vi "Rule_Check_Forbidden.vi"(8 "error in":errorcluster, 9 "Renju":bool=TRUE, 10 "Move":T2={"Row"=7, "Col"=7, "Stone"=enum."Black"}, 11 "Grid":enum8{"Empty", "Black", "White"}[][](array[ring])=[[enum."Empty", enum."Empty", enum."Empty", enum."Empty", enum."Empty", enum."Empty", enum."Empty", enum."Empty", enum."Empty", enum."Empty", enum."Empty", enum."Empty", enum."Empty", enum."Empty", enum."Empty"], [enum."Empty", enum."Empty", enum."Empty", enum."Empty", enum."Empty", enum."Empty", enum."Empty", enum."Empty", enum."Empty", enum."Empty", enum."Empty", enum."Empty", enum."Empty", enum."Empty", enum."Empty"], [enum."Empty", enum."Empty", enum."Empty", enum."Empty", enum."Empty", enum."Empty", enum."Empty", enum."Empty", enum."Empty", enum."Empty", enum."Empty", enum."Empty", enum."Empty", enum."Empty", enum."Empty"], [enum."Empty", enum."Empty", enum."Empty", enum."Empty", enum."Empty", enum."Empty", enum."Empty", enum."Empty", enum."Empty", enum."Empty", enum."Empty", enum."Empty", enum."Empty", enum."Empty", enum."Empty"], [enum."Empty", enum."Empty", enum."Empty", enum."Empty", enum."Empty", enum."Empty", enum."Empty", enum."Empty", enum."Empty", enum."Empty", enum."Empty", enum."Empty", enum."Empty", enum."Empty", enum."Empty"], [enum."Empty", enum."Empty", enum."Empty", enum."Empty", enum."Empty", enum."Empty", enum."Empty", enum."Empty", enum."Empty", enum."Empty", enum."Empty", enum."Empty", enum."Empty", enum."Empty", enum."Empty"], [enum."Empty", enum."Empty", enum."Empty", enum."Empty", enum."Empty", enum."Empty", enum."Empty", enum."Empty", enum."Empty", enum."Empty", enum."Empty", enum."Empty", enum."Empty", enum."Empty", enum."Empty"], [enum."Empty", enum."Empty", enum."Empty", enum."Empty", enum."Empty", enum."Empty", enum."Empty", enum."Empty", enum."Empty", enum."Empty", enum."Empty", enum."Empty", enum."Empty", enum."Empty", enum."Empty"], [enum."Empty", enum."Empty", enum."Empty", enum."Empty", enum."Empty", enum."Empty", enum."Empty", enum."Empty", enum."Empty", enum."Empty", enum."Empty", enum."Empty", enum."Empty", enum."Empty", enum."Empty"], [enum."Empty", enum."Empty", enum."Empty", enum."Empty", enum."Empty", enum."Empty", enum."Empty", enum."Empty", enum."Empty", enum."Empty", enum."Empty", enum."Empty", enum."Empty", enum."Empty", enum."Empty"], [enum."Empty", enum."Empty", enum."Empty", enum."Empty", enum."Empty", enum."Empty", enum."Empty", enum."Empty", enum."Empty", enum."Empty", enum."Empty", enum."Empty", enum."Empty", enum."Empty", enum."Empty"], [enum."Empty", enum."Empty", enum."Empty", enum."Empty", enum."Empty", enum."Empty", enum."Empty", enum."Empty", enum."Empty", enum."Empty", enum."Empty", enum."Empty", enum."Empty", enum."Empty", enum."Empty"], [enum."Empty", enum."Empty", enum."Empty", enum."Empty", enum."Empty", enum."Empty", enum."Empty", enum."Empty", enum."Empty", enum."Empty", enum."Empty", enum."Empty", enum."Empty", enum."Empty", enum."Empty"], [enum."Empty", enum."Empty", enum."Empty", enum."Empty", enum."Empty", enum."Empty", enum."Empty", enum."Empty", enum."Empty", enum."Empty", enum."Empty", enum."Empty", enum."Empty", enum."Empty", enum."Empty"], [enum."Empty", enum."Empty", enum."Empty", enum."Empty", enum."Empty", enum."Empty", enum."Empty", enum."Empty", enum."Empty", enum."Empty", enum."Empty", enum."Empty", enum."Empty", enum."Empty", enum."Empty"]]) -> (0 "error out":errorcluster, 2 "Reason":T1(ring), 3 "Forbidden?":bool)   [LabVIEW 2026]
doc: "렌주룰 흑 금수 판정(3-3, 4-4, 장목). 흑을 가상 착수한 뒤 4방향 연속 수를 본다.\n단순화: 연속된 돌만 판정(띈 3/띈 4 미포함), 거짓 금수 재귀 판정 없음. 정확히 5목이면 금수 아님."
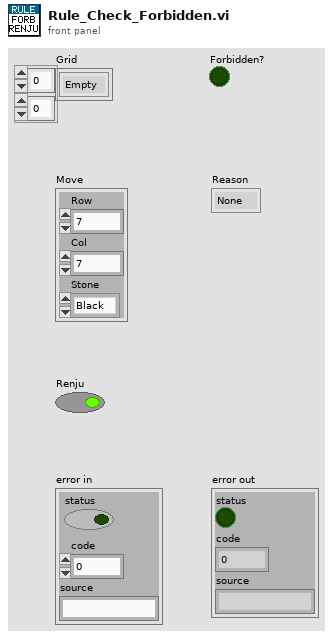
[diagram p1: front panel]
types:
  T1 = enum8{"None", "Double Three", "Double Four", "Overline"}
  T2 = cluster{"Row":i32, "Col":i32, "Stone":enum8{"Empty", "Black", "White"}}
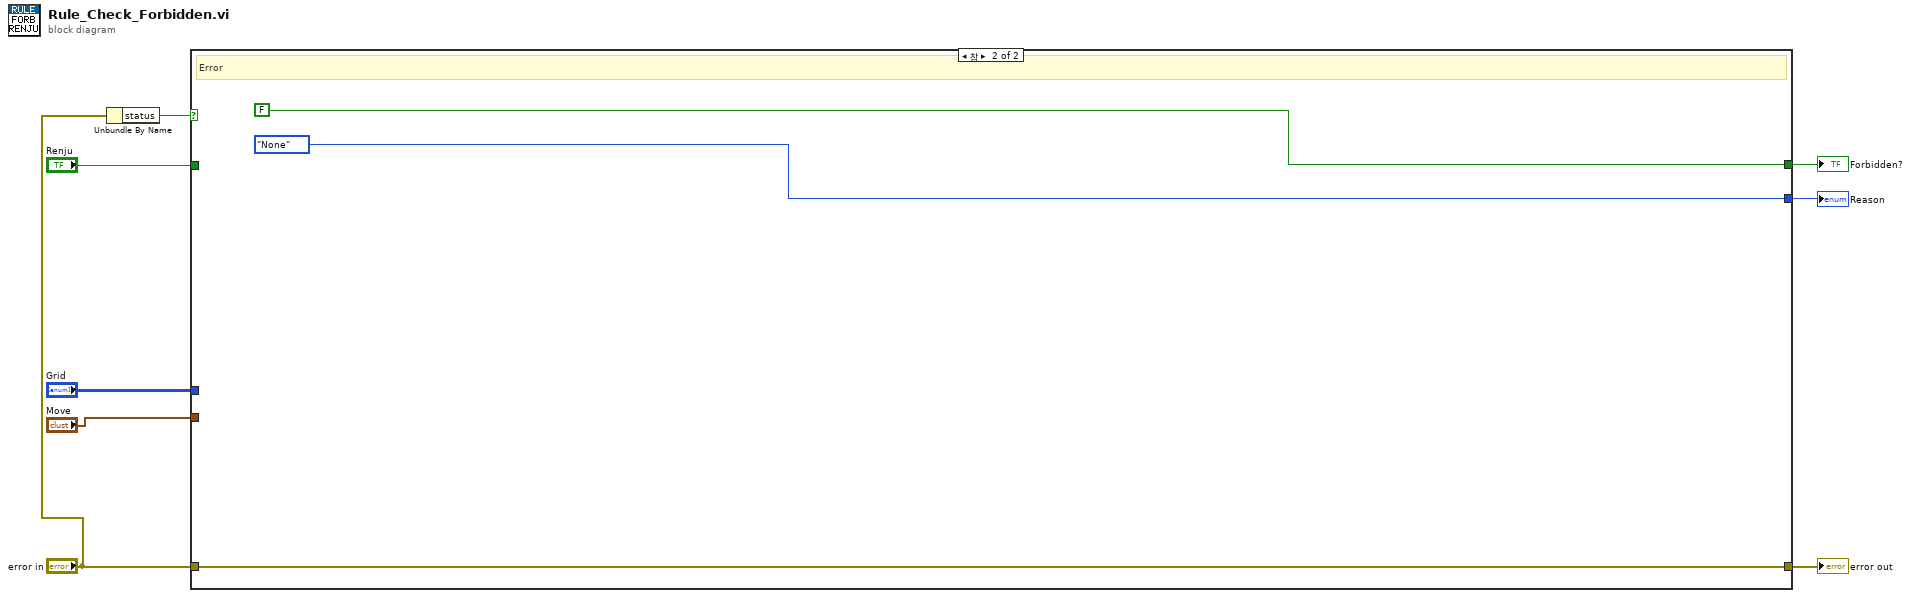
[diagram p0: block diagram]
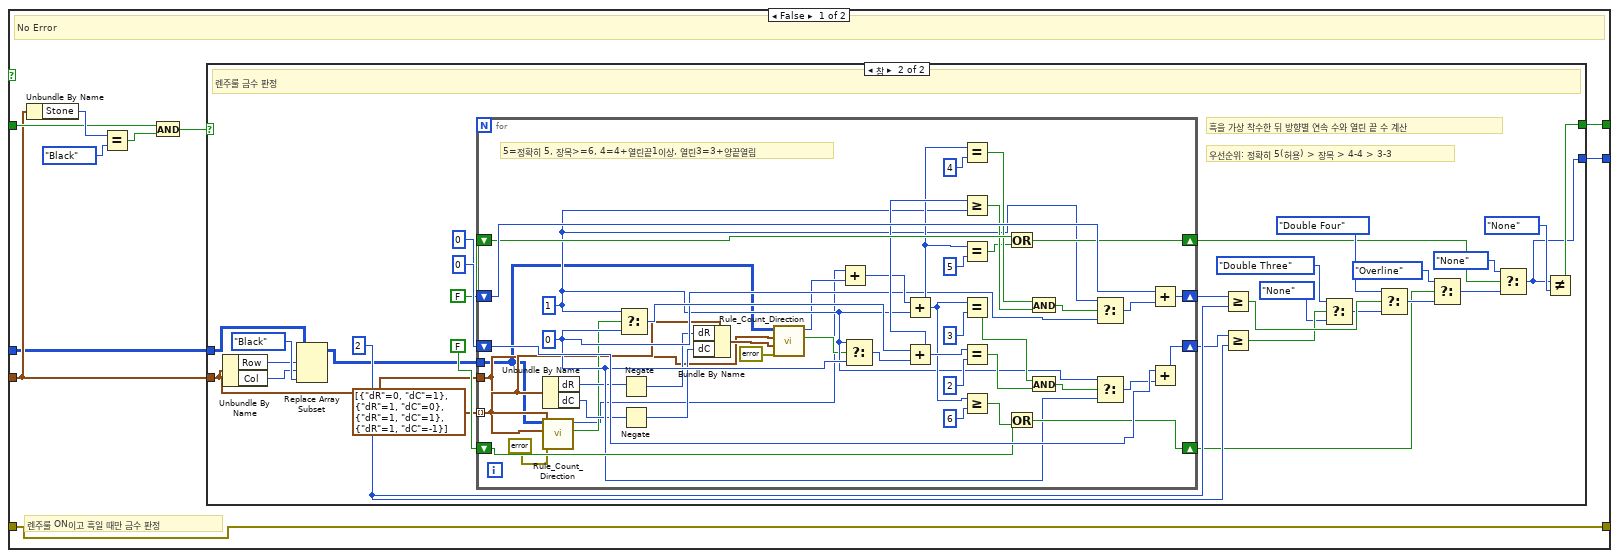
[diagram p2: hidden frame]
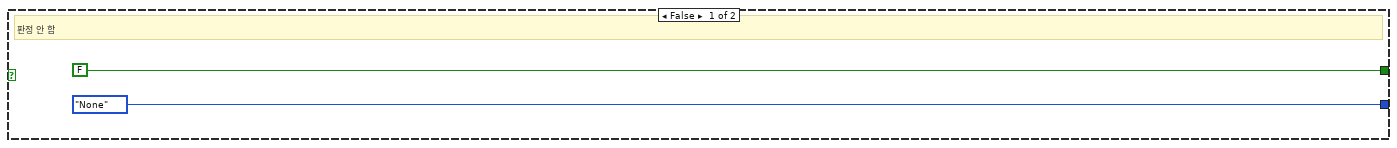
[diagram p3: hidden frame]
diagram:
  n1 = Unbundle By Name("error in") -> ("status"=w5:bool)
  n2 = case shown="참" w5 {
    tunnel: "Grid" -> [w9 _]
    tunnel: "Move" -> [w10 _]
    tunnel: "Renju" -> [w11 _]
    tunnel: "error in" -> [w12 w94]
    tunnel: [w12 w94] -> w8
    tunnel: [w18 T1."None"] -> w7
    tunnel: [w17 FALSE] -> w6
    frame False {
      # "렌주룰 ON이고 흑일 때만 금수 판정"
      # "No Error"
      n3 = Unbundle By Name(w10) -> ("Stone"=w13:enum8{"Empty", "Black", "White"})
      n4 = Equal?(x=w13, y=enum8{"Empty", "Black", "White"}."Black") -> (x = y?=w15:bool)
      n5 = And(x=w11, y=w15) -> (x .and. y?=w16:bool)
      n6 = case shown="참" w16 {
        tunnel: w9 -> [_ w21]
        tunnel: w10 -> [_ w22]
        tunnel: [T1."None" w47] -> w18
        tunnel: [FALSE w49] -> w17
        frame False {
          # "판정 안 함"
        }
        frame True {
          w36 = 2
          # "우선순위: 정확히 5(허용) > 장목 > 4-4 > 3-3"
          # "흑을 가상 착수한 뒤 방향별 연속 수와 열린 끝 수 계산"
          # "렌주룰 금수 판정"
          n7 = Unbundle By Name(w22) -> ("Row"=w23:i32, "Col"=w24:i32)
          n8 = Replace Array Subset(array=w21, new element=enum8{"Empty", "Black", "White"}."Black", index (row)=w23, index (col)=w24) -> (w26:enum8{"Empty", "Black", "White"}[][])
          n9 = for {
            tunnel: cluster{"dR":i32, "dC":i32}[] [{"dR"=0, "dC"=1}, {"dR"=1, "dC"=0}, {"dR"=1, "dC"=1}, {"dR"=1, "dC"=-1}] ("Directions") -> [w52] mode=indexing
            shift-right: [w84] -> w32
            shift-left: FALSE -> [w85]
            shift-right: [w86] -> w33
            shift-left: FALSE -> [w87]
            shift-right: [w89] -> w34
            shift-left: 0 -> [w90]
            shift-right: [w92] -> w35
            shift-left: 0 -> [w93]
            tunnel: w22 -> [w51]
            tunnel: w26 -> [w50]
            w65 = 0
            w64 = 1
            # "5=정확히 5, 장목>=6, 4=4+열린끝1이상, 열린3=3+양끝열림"
            n10 = Unbundle By Name(w52) -> ("dR"=w56:i32, "dC"=w57:i32)
            n11 = call "Rule_Count_Direction.vi"("error in"=errorcluster {"status"=FALSE, "code"=0, "source"=""}, "Direction"=w52, "Move"=w51, "Grid"=w50) -> ("Open End"=w55:bool, "Count"=w54:i32)  [unwired: 5 in, 1 out]
            n12 = Select(t=w64, s=w55, f=w65) -> (s? t:f=w68:i32)
            n13 = Negate(x=w56) -> (-x=w58:i32)
            n14 = Negate(x=w57) -> (-x=w59:i32)
            n15 = Bundle By Name(cluster=w52, "dR"=w58, "dC"=w59) -> (w60:cluster{"dR":i32, "dC":i32})
            n16 = call "Rule_Count_Direction.vi"("error in"=errorcluster {"status"=FALSE, "code"=0, "source"=""}, "Direction"=w60, "Move"=w51, "Grid"=w50) -> ("Open End"=w63:bool, "Count"=w62:i32)  [unwired: 5 in, 1 out]
            n17 = Add(x=w54, y=w62) -> (x+y=w66:i32)
            n18 = Select(t=w64, s=w63, f=w65) -> (s? t:f=w69:i32)
            n19 = Add(x=w66, y=w64) -> (x+y=w67:i32)
            n20 = Add(x=w68, y=w69) -> (x+y=w70:i32)
            n21 = Equal?(x=w67, y=4) -> (x = y?=w76:bool)
            n22 = Greater Or Equal?(x=w70, y=w64) -> (x >= y?=w77:bool)
            n23 = Equal?(x=w67, y=5) -> (x = y?=w72:bool)
            n24 = Equal?(x=w67, y=3) -> (x = y?=w80:bool)
            n25 = Equal?(x=w70, y=2) -> (x = y?=w82:bool)
            n26 = Greater Or Equal?(x=w67, y=6) -> (x >= y?=w74:bool)
            n27 = Or(x=w85, y=w72) -> (x .or. y?=w84:bool)
            n28 = Or(x=w87, y=w74) -> (x .or. y?=w86:bool)
            n29 = And(x=w76, y=w77) -> (x .and. y?=w78:bool)
            n30 = And(x=w80, y=w82) -> (x .and. y?=w83:bool)
            n31 = Select(t=w64, s=w78, f=w65) -> (s? t:f=w88:i32)
            n32 = Select(t=w64, s=w83, f=w65) -> (s? t:f=w91:i32)
            n33 = Add(x=w90, y=w88) -> (x+y=w89:i32)
            n34 = Add(x=w93, y=w91) -> (x+y=w92:i32)
          }
          n35 = Greater Or Equal?(x=w34, y=w36) -> (x >= y?=w43:bool)
          n36 = Greater Or Equal?(x=w35, y=w36) -> (x >= y?=w41:bool)
          n37 = Select(t=T1."Double Three", s=w41, f=T1."None") -> (s? t:f=w42:T1)
          n38 = Select(t=T1."Double Four", s=w43, f=w42) -> (s? t:f=w44:T1)
          n39 = Select(t=T1."Overline", s=w33, f=w44) -> (s? t:f=w45:T1)
          n40 = Select(t=T1."None", s=w32, f=w45) -> (s? t:f=w47:T1)
          n41 = Not Equal?(x=w47, y=T1."None") -> (x != y?=w49:bool)
        }
      }
    }
    frame True {
      # "Error"
    }
  }
  "Forbidden?" <- w6
  "Reason" <- w7
  "error out" <- w8
